vi "Generate Paths And Strings.vi"(10 "Python Module":path, 11 "Output Folder":path) -> (3 "Paths":T1)   [LabVIEW 2026]
doc: "Generate paths and strings from input paths."
uses:
  Paths And Strings--cluster.ctl
  <userlib>/_OpenG.lib/file/file.llb/Strip Path - Traditional__ogtk.vi
  <userlib>/_OpenG.lib/file/file.llb/Strip Path Extension - String__ogtk.vi
  <userlib>/_OpenG.lib/file/file.llb/Convert File Extension (String)__ogtk.vi
  <userlib>/_OpenG.lib/file/file.llb/openg_file.lvlib
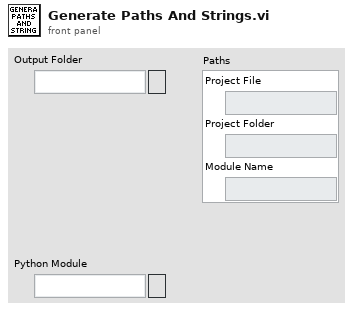
[diagram p1: front panel]
types:
  T1 = typedef "Paths And Strings--cluster.ctl" = cluster{"Project File":path, "Project Folder":path, "Module Name":string}
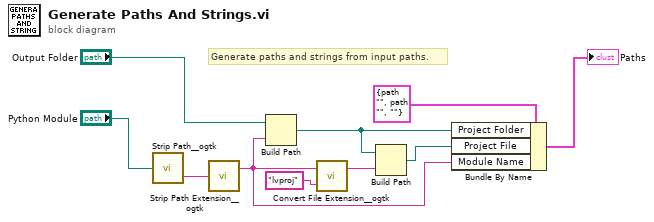
[diagram p0: block diagram]
diagram:
  # "Generate paths and strings from input paths."
  n1 = call-poly <userlib>:"Strip Path__ogtk.vi"("path"="Python Module") -> ("name"=w9:string)  [unwired: 1 out]
  n2 = call-poly <userlib>:"Strip Path Extension__ogtk.vi"("path"=w9) -> ("root"=w2:string)  [unwired: 1 out]
  n3 = Build Path(base path="Output Folder", name or relative path=w2) -> (appended path=w5:path)
  n4 = call-poly <userlib>:"Convert File Extension__ogtk.vi"("new ending (none)"="lvproj", "file name"=w2) -> ("new filename"=w4:string)  [unwired: 1 out]
  n5 = Build Path(base path=w5, name or relative path=w4) -> (appended path=w3:path)
  n6 = Bundle By Name(cluster=T1 {"Project File"=path "", "Project Folder"=path "", "Module Name"=""} ("Paths"), "Project Folder"=w5, "Project File"=w3, "Module Name"=w2) -> (→"Paths":T1)
